vi "Configure SM.vi"(8 "error in (no error)":errorcluster, 9 "Sweep start V":dbl, 10 "Protection C":dbl, 11 "Puerto serial":refnum<visa-resource-name>) -> (0 "error out":errorcluster)   [LabVIEW 2020]
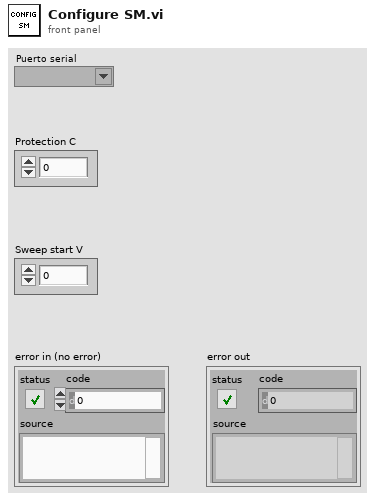
[diagram p1: front panel]
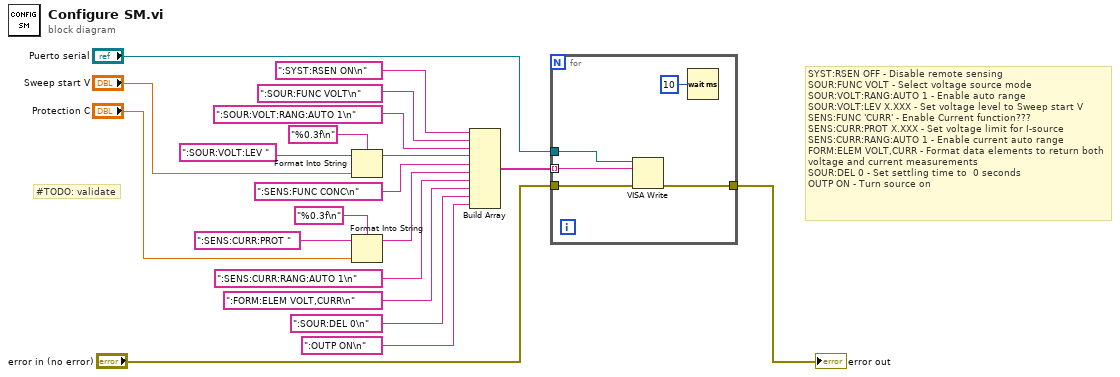
[diagram p0: block diagram]
diagram:
  # "#TODO: validate"
  # "SYST:RSEN OFF - Disable remote sensing\nSOUR:FUNC VOLT - Select voltage source mode\nSOUR:VOLT:RANG:AUTO 1 - Enable auto range \nSOUR:VOLT:LEV X.XXX - Set voltage level to Sweep start V \nSENS:FUNC 'CURR' - Enable Current function??? \nSENS:CURR:PROT X.XXX - Set voltage limit for I-source \nSENS:CURR:RANG:AUTO 1 - Enable current auto range \nFORM:ELEM VOLT,CURR - Format data elements to return both voltage and current measurements  \nSOUR:DEL 0 - Set settling time to  0 seconds\nOUTP ON - Turn source on"
  n1 = Format Into String(format string="%0.3f\n", initial string=":SOUR:VOLT:LEV " ("Comando"), "Sweep start V") -> (resulting string=w10:string)  [unwired: 1 in, 1 out]
  n2 = Format Into String(format string="%0.3f\n", initial string=":SENS:CURR:PROT " ("Comando"), "Protection C") -> (resulting string=w8:string)  [unwired: 1 in, 1 out]
  n3 = Build Array(":SYST:RSEN ON\n" ("Comando"), ":SOUR:FUNC VOLT\n" ("Comando"), ":SOUR:VOLT:RANG:AUTO 1\n" ("Comando"), w10, ":SENS:FUNC CONC\n" ("Comando"), w8, ":SENS:CURR:RANG:AUTO 1\n" ("Comando"), ":FORM:ELEM VOLT,CURR\n" ("Comando"), ":SOUR:DEL 0\n" ("Comando"), ":OUTP ON\n" ("Comando")) -> (w3:string[])
  n4 = for {
    tunnel: "Puerto serial" -> [w23]
    tunnel: w3 -> [w22] mode=indexing
    tunnel: "error in (no error)" -> [w25]
    tunnel: [w24] -> w1
    n5 = VISA Write(VISA resource name=w23, write buffer=w22, error in (no error)=w25) -> (error out=w24:errorcluster)  [unwired: 2 out]
    n6 = Wait (ms)(milliseconds to wait=u32 10) -> ()  [unwired: 1 out]
  }
  "error out" <- w1
